vi "VIH HelpGen - Palette - Convert NI Palette Items to VIH Items Info.vi"(8 "error in":errorcluster, 9 "Palette Items":T3, 11 "Palette Path":path) -> (0 "error out":errorcluster, 1 "Items Array":T1[](array[typedef]), 3 "dup Palette Path":path)   [LabVIEW 2014]
doc: "::: VI Helpeks :::\nCopyright (c) 2000-2026 Konstantin Shifershteyn. All rights reserved."
uses:
  <vilib>/Palette API/Palette Menu/Public Type Define/Items.ctl
  <vilib>/Palette API/Palette Menu/Public Type Define/Item.ctl
  VIH HelpGen Typedef - Palette - Item Info Cluster.ctl
  VIH HelpGen Typedef - Palette - Item Type Enum.ctl
  <vilib>/Palette API/Palette Menu/Palette Menu.lvlib
panel:
  # "VI Helpeks\nCopyright (c) 2012-2026 Konstantin Shifershteyn"
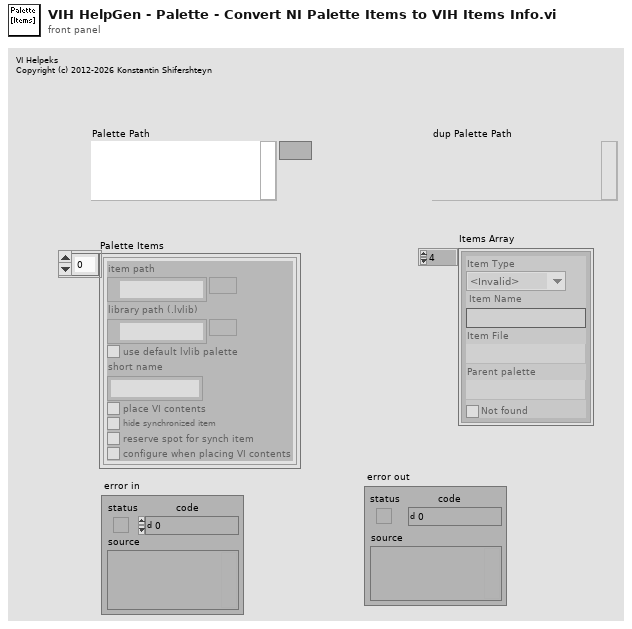
[diagram p1: front panel]
types:
  T1 = typedef "VIH HelpGen Typedef - Palette - Item Info Cluster.ctl" = cluster{"Item Type":T2, "Item Name":string, "Item File":path, "Parent palette":path, "Not found":bool}
  T2 = typedef "VIH HelpGen Typedef - Palette - Item Type Enum.ctl" = enum32{"<Invalid>", "<unknown>", "VI", "Menu", "LV Func", "Express VI", "Poly VI", "CTL", "HTML"}
  T3 = typedef "Palette Menu.lvlib/Items.ctl" = T4[]
  T4 = typedef "Palette Menu.lvlib/Item.ctl" = cluster{"item path":path, "library path (.lvlib)":path, "use default lvlib palette":bool, "short name":string, "place VI contents":bool, "hide synchronized item":bool, "reserve spot for synch item":bool, "configure when placing VI contents":bool}
  T5 = typedef "Palette Menu.lvlib/Palette Data.ctl" = cluster{"display name":string, "view format":T6, "palette width":i16, "items":T3, "256 color icon":picture, "B&W color icon":picture, "help information":T7, "palette description":string, "synchronize information":T8}
  T6 = typedef "Palette Menu.lvlib/View Format.ctl" = u16
  T7 = typedef "Palette Menu.lvlib/Help Info.ctl" = cluster{"help tag":string, "help file path ":path}
  T8 = typedef "Palette Menu.lvlib/Synchronize Info.ctl" = cluster{"synchronize with directory":bool, "synchronize directory path":path}
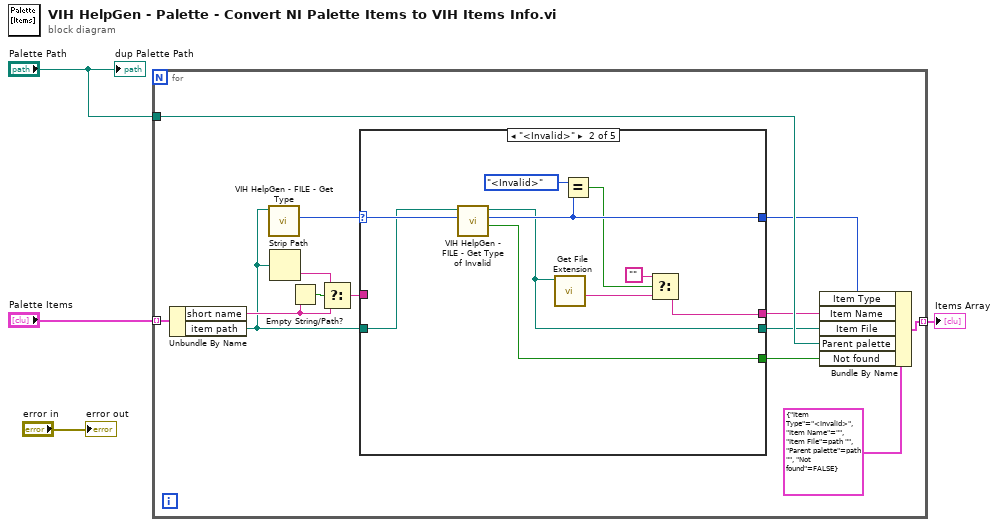
[diagram p0: block diagram]
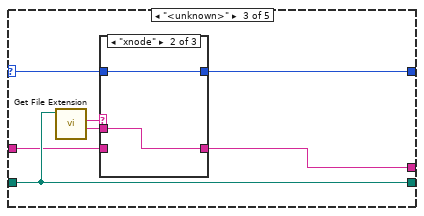
[diagram p3: hidden frame]
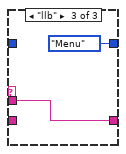
[diagram p5: hidden frame]
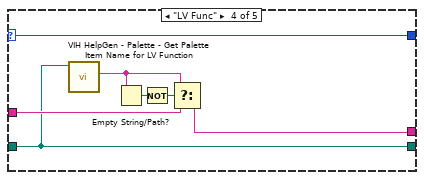
[diagram p6: hidden frame]
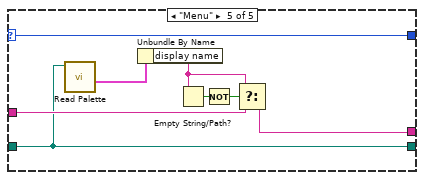
[diagram p7: hidden frame]
diagram:
  n1 = for {
    tunnel: [w18] -> w3 mode=indexing
    tunnel: "Palette Path" -> [w17]
    tunnel: "Palette Items" -> [w16] mode=indexing
    n2 = Unbundle By Name(w16) -> ("short name"=w15:string, "item path"=w10:path)
    n3 = call "VIH HelpGen - FILE - Get Type.vi"("File Path"=w10) -> ("File Type"=w9:T2)  [unwired: 8 in, 2 out]
    n4 = Strip Path(path=w10) -> (name=w5:string)  [unwired: 1 out]
    n5 = Empty String/Path?(string/path=w15) -> (empty?=w14:bool)
    n6 = Select(t=w5, s=w14, f=w15) -> (s? t:f=w13:string)
    n7 = case shown="\"<Invalid>\"" w9 {
      selector: w9 -> [w19 w31 w32 w46 w53]
      tunnel: w13 -> [w21 _ w35 w48 w55]
      tunnel: [w21 w28 w36 w50 w54] -> w12
      tunnel: [w20 w22 w38 w45 w52] -> w11
      tunnel: w10 -> [w20 w30 w38 w45 w52]
      tunnel: [w19 w25 w33 w46 w53] -> w7
      tunnel: [_ w29 _ _ _] -> w6
      frame Default {
      }
      frame "<Invalid>" {
        n8 = call "VIH HelpGen - FILE - Get Type of Invalid.vi"("File Type"=w31, "File Path"=w30) -> ("Not found"=w29:bool, "File Type out"=w25:T2, "File Path out"=w22:path)  [unwired: 6 in, 1 out]
        n9 = call <vilib>:"Get File Extension.vi"("file"=w22) -> ("filename without extension"=w23:string)  [unwired: 7 in, 3 out]
        n10 = Equal?(x=VIH_HelpGen_Typedef_-_Palette_-_Item_Type_Enum."<Invalid>", y=w25) -> (x = y?=w24:bool)
        n11 = Select(t="", s=w24, f=w23) -> (s? t:f=w28:string)
      }
      frame "<unknown>" {
        n12 = call <vilib>:"Get File Extension.vi"("file"=w38) -> ("filename without extension"=w34:string, "lowercase file extension"=w37:string)  [unwired: 7 in, 2 out]
        n13 = case shown="\"xnode\"" w37 {
          tunnel: [w40 w42 w44] -> w36
          tunnel: w35 -> [w40 _ _]
          tunnel: w34 -> [_ w42 w44]
          tunnel: [w39 w41 VIH_HelpGen_Typedef_-_Palette_-_Item_Type_Enum."Menu" ("File Type")] -> w33
          tunnel: w32 -> [w39 w41 _]
          frame Default {
          }
          frame "xnode" {
          }
          frame "llb" {
          }
        }
      }
      frame "LV Func" {
        n14 = call "VIH HelpGen - Palette - Get Palette Item Name for LV Function.vi"("Path"=w45) -> ("Name"=w47:string)  [unwired: 8 in, 2 out]
        n15 = Empty String/Path?(string/path=w47) -> (empty?=w51:bool)
        n16 = Not(x=w51) -> (.not. x?=w49:bool)
        n17 = Select(t=w47, s=w49, f=w48) -> (s? t:f=w50:string)
      }
      frame "Menu" {
        n18 = call <vilib>:"Read Palette.vi"("palette path"=w52) -> ("palette data"=w59:T5)  [unwired: 8 in, 2 out]
        n19 = Unbundle By Name(w59) -> ("display name"=w56:string)
        n20 = Empty String/Path?(string/path=w56) -> (empty?=w58:bool)
        n21 = Not(x=w58) -> (.not. x?=w57:bool)
        n22 = Select(t=w56, s=w57, f=w55) -> (s? t:f=w54:string)
      }
    }
    n23 = Bundle By Name(cluster=T1 {"Item Type"=enum."<Invalid>", "Item Name"="", "Item File"=path "", "Parent palette"=path "", "Not found"=FALSE} ("Item Info"), "Item Type"=w7, "Item Name"=w12, "Item File"=w11, "Parent palette"=w17, "Not found"=w6) -> (w18:T1)
  }
  "Items Array" <- w3
  "error out" <- "error in"
  "dup Palette Path" <- "Palette Path"
